vi "Create deserializer.vi"(0 "VI in":refnum<vi>, 5 "Terms[]":refnum<vi>[](array[refnum]), 7 "Control Names Out":string[](array[string]), 11 "error in (no error)":errorcluster) -> (15 "error out":errorcluster)   [LabVIEW 2021, in "Migrator.lvlib"]
uses:
  Migrator.lvlib
  <vilib>/Utility/miscctls.llb/LVPointTypeDef.ctl
  Path Functions/Path Functions.lvlib
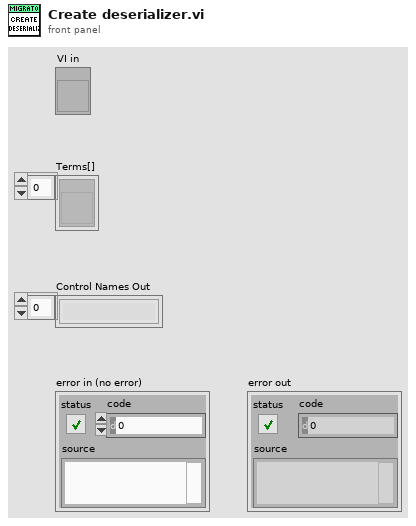
[diagram p1: front panel]
types:
  T1 = typedef "LVPointTypeDef.ctl" = cluster{"Horizontal":i16, "Vertical":i16}
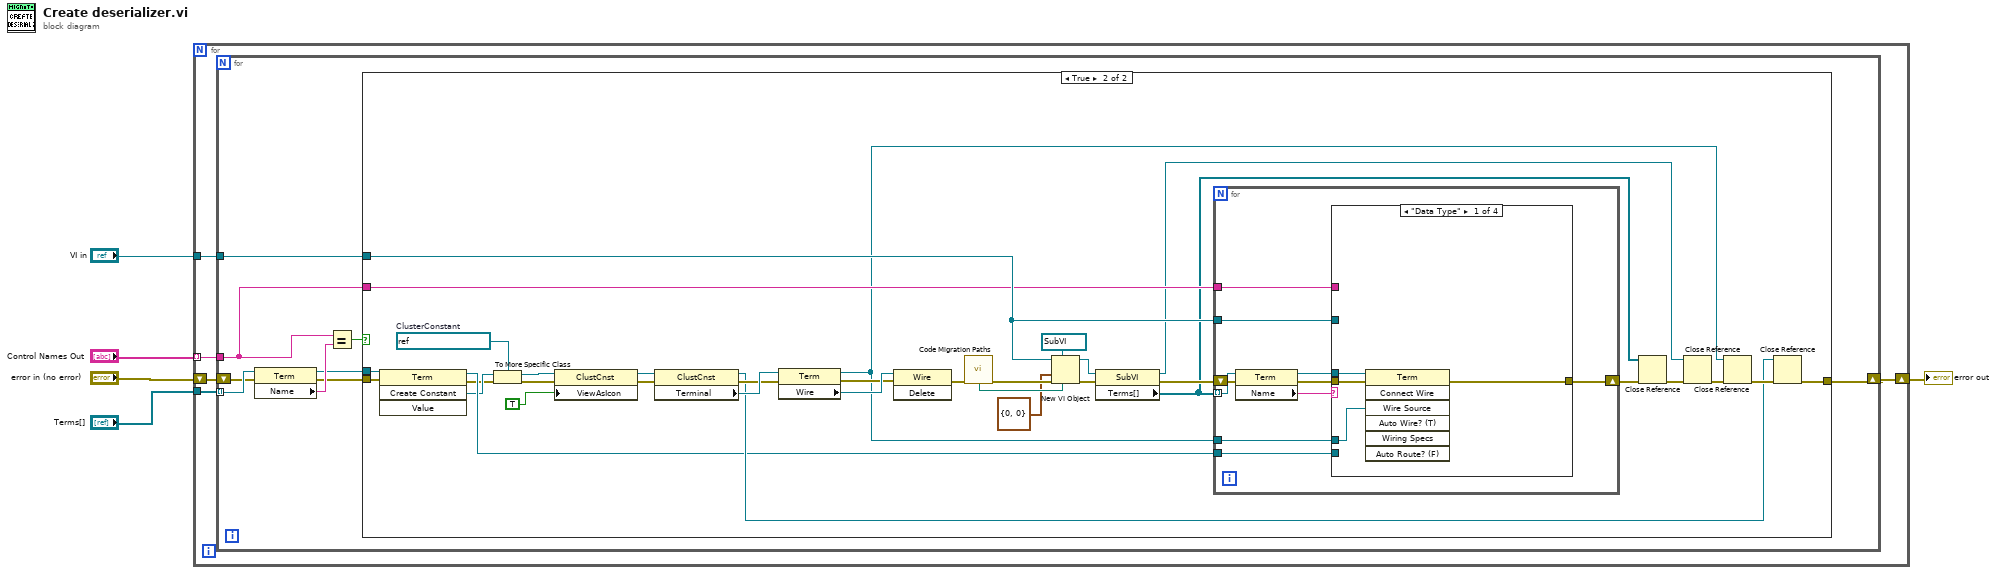
[diagram p0: block diagram]
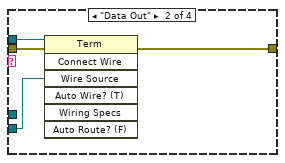
[diagram p3: hidden frame]
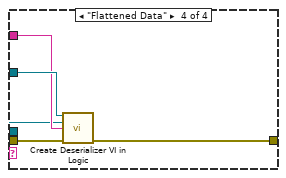
[diagram p5: hidden frame]
diagram:
  n1 = for {
    tunnel: "Terms[]" -> [w10]
    tunnel: "Control Names Out" -> [w8] mode=indexing
    shift-right: [w6] -> w4
    shift-left: "error in (no error)" -> [w9]
    tunnel: "VI in" -> [w7]
    n2 = for {
      tunnel: w10 -> [w19] mode=indexing
      shift-right: [w12] -> w6
      shift-left: w9 -> [w17]
      tunnel: w8 -> [w11]
      tunnel: w7 -> [w13]
      n3 = property class="Term"(reference=w19, error in=w17) -> (reference out=w14:refnum<vi>, error out=w15:errorcluster, "Name"=w18:string)
      n4 = Equal?(x=w11, y=w18) -> (x = y?=w16:bool)
      n5 = case shown="True" w16 {
        tunnel: w15 -> [w20 w53]
        tunnel: w14 -> [_ w54]
        tunnel: w13 -> [_ w40]
        tunnel: [w20 w31] -> w12
        tunnel: w11 -> [_ w39]
        frame False {
        }
        frame True {
          w26 = refnum<vi> refnum  # ClusterConstant
          n6 = invoke class="Term" method="Create Constant"(reference=w54, error in=w53) -> (reference out=w30:refnum<vi>, error out=w24:errorcluster, "Create Constant"=w28:refnum<vi>)  [unwired: 2 in, 1 out]
          n7 = To More Specific Class(target class=w26, reference=w28, error in=w24) -> (specific class reference=w27:refnum<vi>, error out=w23:errorcluster)
          n8 = property class="ClustCnst"(reference=w27, error in=w23, "ViewAsIcon"=TRUE ("View As Icon")) -> (reference out=w22:refnum<vi>, error out=w21:errorcluster)
          n9 = property class="ClustCnst"(reference=w22, error in=w21) -> (reference out=w32:refnum<vi>, error out=w42:errorcluster, "Terminal"=w44:refnum<vi>)
          n10 = property class="Term"(reference=w44, error in=w42) -> (reference out=w29:refnum<vi>, error out=w41:errorcluster, "Wire"=w43:refnum<vi>)
          n11 = invoke class="Wire" method="Delete"(reference=w43, error in=w41) -> (error out=w52:errorcluster)  [unwired: 1 in, 2 out]
          n12 = call "Code Migration Paths.vi"("error in (no error)"=w52) -> ("Deserializer"=w51:path, "error out"=w50:errorcluster)  [unwired: 7 in, 6 out]
          n13 = New VI Object(vi object class=refnum<vi> refnum ("Other Refnum"), owner refnum=w40, position/next to=T1 {"Horizontal"=0, "Vertical"=0} ("location"), 6:w51, 8:w50) -> (object refnum=w47:refnum<vi>, 0:w46:errorcluster)  [unwired: 3 in]
          n14 = property class="SubVI"(reference=w47, error in=w46) -> (reference out=w35:refnum<vi>, error out=w45:errorcluster, "Terms[]"=w37:refnum<vi>[])
          n15 = for {
            tunnel: w37 -> [w61] mode=indexing
            shift-right: [w59] -> w38
            shift-left: w45 -> [w64]
            tunnel: w40 -> [w58]
            tunnel: w39 -> [w57]
            tunnel: w30 -> [w56]
            tunnel: w29 -> [w55]
            n16 = property class="Term"(reference=w61, error in=w64) -> (reference out=w60:refnum<vi>, error out=w63:errorcluster, "Name"=w62:string)
            n17 = case shown="\"Data Type\"" w62 {
              tunnel: w63 -> [w67 w72 w73 w78]
              tunnel: w60 -> [w68 w71 _ w75]
              tunnel: [w66 w70 w73 w74] -> w59
              tunnel: w58 -> [_ _ _ w77]
              tunnel: w57 -> [_ _ _ w76]
              tunnel: w56 -> [_ w69 _ _]
              tunnel: w55 -> [w65 _ _ _]
              frame "Data Type" {
                n18 = invoke class="Term" method="Connect Wire"(reference=w68, error in=w67, "Wire Source"=w65) -> (error out=w66:errorcluster)  [unwired: 4 in, 6 out]
              }
              frame "Data Out" {
                n19 = invoke class="Term" method="Connect Wire"(reference=w71, error in=w72, "Wire Source"=w69) -> (error out=w70:errorcluster)  [unwired: 4 in, 6 out]
              }
              frame Default {
              }
              frame "Flattened Data" {
                n20 = call "Create Deserializer VI in Logic.vi"("VI in"=w77, "Term Refnum"=w75, "Name Out"=w76, "error in (no error)"=w78) -> ("error out"=w74:errorcluster)  [unwired: 11 in]
              }
            }
          }
          n21 = Close Reference(reference=w37, error in (no error)=w38) -> (error out=w36:errorcluster)
          n22 = Close Reference(reference=w35, error in (no error)=w36) -> (error out=w34:errorcluster)
          n23 = Close Reference(reference=w29, error in (no error)=w34) -> (error out=w33:errorcluster)
          n24 = Close Reference(reference=w32, error in (no error)=w33) -> (error out=w31:errorcluster)
        }
      }
    }
  }
  "error out" <- w4
